vi "VI Helpeks API Example.vi"   [LabVIEW 2014]
doc: "::: VI Helpeks :::\nCopyright (c) 2000-2026 Konstantin Shifershteyn. All rights reserved."
panel:
  # "Opening VI Helpeks API Example..."
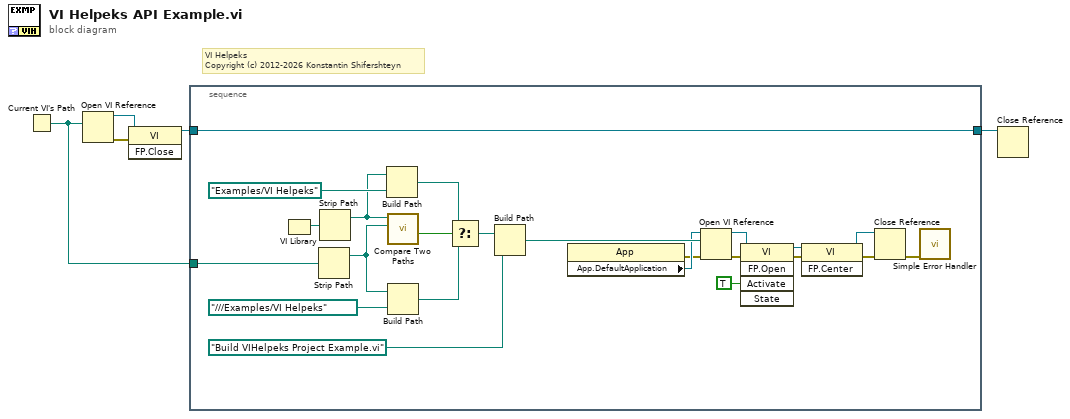
[diagram p0: block diagram]
diagram:
  # "VI Helpeks\nCopyright (c) 2012-2026 Konstantin Shifershteyn"
  n1 = Current VI's Path() -> (path=w1:path)
  n2 = Open VI Reference(vi path=w1) -> (vi reference=w4:refnum<vi>, error out=w5:errorcluster)  [unwired: 5 in]
  n3 = invoke class="VI" method="FP.Close"(reference=w4, error in=w5) -> (reference out=w3:refnum<vi>)  [unwired: 1 in, 2 out]
  n4 = stacked-sequence {
    tunnel: [w28] -> w2
    tunnel: w3 -> [w28]
    tunnel: w1 -> [w17]
    frame #0 {
      n5 = VI Library() -> (path=w18:path)
      n6 = Strip Path(path=w17) -> (stripped path=w25:path)  [unwired: 1 out]
      n7 = Strip Path(path=w18) -> (stripped path=w20:path)  [unwired: 1 out]
      n8 = Build Path(base path=w20, name or relative path=path "Examples/VI Helpeks") -> (appended path=w22:path)
      n9 = call <vilib>:"Compare Two Paths.vi"("Path 2"=w25, "Path 1"=w20) -> ("Path 2 Relative to Path 1?"=w19:bool)  [unwired: 6 in, 3 out]
      n10 = Build Path(base path=w25, name or relative path=path "../../../Examples/VI Helpeks") -> (appended path=w27:path)
      n11 = Select(t=w22, s=w19, f=w27) -> (s? t:f=w21:path)
      n12 = Build Path(base path=w21, name or relative path=path "Build VIHelpeks Project Example.vi" ("append path")) -> (appended path=w16:path)
      n13 = property class="App"() -> (error out=w6:errorcluster, "App.DefaultApplication"=w8:refnum<vi>)  [unwired: 2 in, 1 out]
      n14 = Open VI Reference(application reference (local)=w8, vi path=w16, error in (no error)=w6) -> (vi reference=w14:refnum<vi>, error out=w15:errorcluster)  [unwired: 3 in]
      n15 = invoke class="VI" method="FP.Open"(reference=w14, error in=w15, "Activate"=TRUE ("Activate?")) -> (reference out=w11:refnum<vi>, error out=w12:errorcluster)  [unwired: 2 in, 3 out]
      n16 = invoke class="VI" method="FP.Center"(reference=w11, error in=w12) -> (reference out=w9:refnum<vi>, error out=w10:errorcluster)  [unwired: 1 in, 1 out]
      n17 = Close Reference(reference=w9, error in (no error)=w10) -> (error out=w7:errorcluster)
      n18 = call <vilib>:"Simple Error Handler.vi"("error in (no error)"=w7) -> ()  [unwired: 4 in, 5 out]
    }
  }
  n19 = Close Reference(reference=w2) -> ()  [unwired: 1 in, 1 out]
